vi "CSM - Revert Arguments-Safe String.vi"(2 "Safe Argument String":string="eaasdf->fqwvrf", 4 "Force Convert (F)":bool) -> (7 "Origin Argument String":string)   [LabVIEW 2017, in "Communicable State Machine.lvlib"]
doc: "Converts the %Hex format CSM keywords in the safe string argument back to the original format.\n\n- When <b>Force Convert (F)</b> is FALSE, conversion is performed only if the argument type tag is `SAFESTR`.\n- When <b>Force Convert (F)</b> is TRUE, conversion is performed regardless of the argument type tag.\n\n\n> [!NOTE] <b>CSM Message Keywords</b>\n>\n> The following are CSM message keywords: `->`, `->|`, `-@`, `-&`, `<-`, `\\r`, `\\n`, `//`, `>>`, `>>>`, `>>>>`, `;`, `,`.\n\n\n> [!NOTE] <b>CSM Safe String Argument</b>\n>\n> To pass arbitrary strings in CSM arguments without disrupting message parsing, CSM has a built-in Safe-String encoding/decoding scheme. The argument type string is SAFESTR. The conversion process is as follows:\n> 1. Scan the input string. If any CSM keywords, such as `->`, `;`, `\\r` appear, replace them with `%Hex` escape sequences.\n> 2. Obtain the argument in the form `<SAFESTR> escaped string`, which can be safely embedded in the state string without disrupting CSM message parsing.\n\n\n<b>Reference Example</b>: `[CSM-Example]\\0. Base Concepts\\4.3 Arguments - Safe Arguments if it contains key words of CSM.vi`.\n\n-- <b>Controls</b> --\n- <b>Safe Argument String</b>: Safe string argument.\n- <b>Force Convert (F)</b>: Force conversion, even if the argument type tag is not `SAFESTR`.\n\n-- <b>Indicators</b> --\n- <b>Origin Argument String</b>: String argument."
uses:
  Communicable State Machine.lvlib
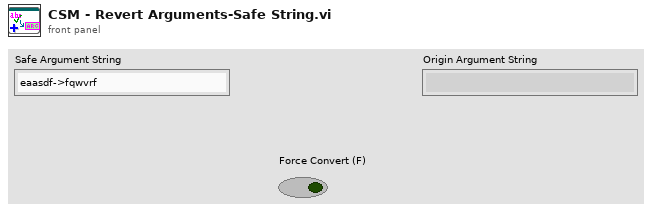
[diagram p1: front panel]
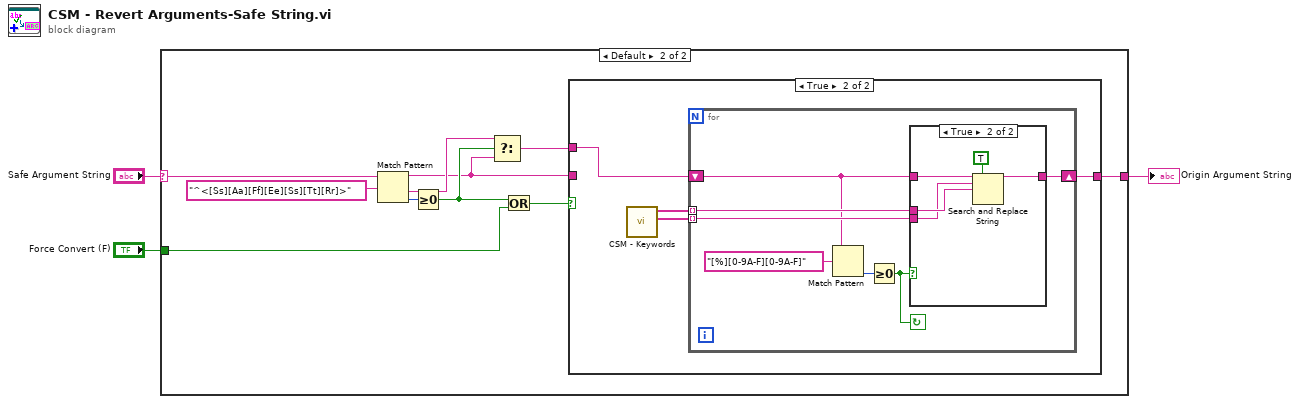
[diagram p0: block diagram]
diagram:
  n1 = case shown="Default" "Safe Argument String" {
    selector: "Safe Argument String" -> [w4 w11]
    tunnel: [w4 w14] -> w2
    tunnel: "Force Convert (F)" -> [_ w9]
    frame "" {
    }
    frame Default {
      n2 = Match Pattern(string=w11, regular expression="^<[Ss][Aa][Ff][Ee][Ss][Tt][Rr]>") -> (before substring=w6:string, after substring=w7:string, offset past match=w12:i32)  [unwired: 1 in, 1 out]
      n3 = Greater Or Equal To 0?(x=w12) -> (x >= 0?=w8:bool)
      n4 = Select(t=w7, s=w8, f=w6) -> (s? t:f=w5:string)
      n5 = Or(x=w8, y=w9) -> (x .or. y?=w10:bool)
      n6 = case shown="True" w10 {
        tunnel: [w15 w19] -> w14
        tunnel: w6 -> [w15 _]
        tunnel: w5 -> [_ w16]
        frame False {
        }
        frame True {
          n7 = call "CSM - Keywords.vi"() -> ("Keywords (%Hex Format)"=w18:string[], "Keywords"=w17:string[])  [unwired: 10 in]
          n8 = for {
            shift-right: [w26] -> w19
            shift-left: w16 -> [w23]
            tunnel: w17 -> [w25] mode=indexing
            tunnel: w18 -> [w24] mode=indexing
            stop <- w20 continue-if-true
            n9 = Match Pattern(string=w23, regular expression="[%][0-9A-F][0-9A-F]") -> (offset past match=w21:i32)  [unwired: 1 in, 3 out]
            n10 = Greater Or Equal To 0?(x=w21) -> (x >= 0?=w20:bool)
            n11 = case shown="True" w20 {
              tunnel: [w27 w31] -> w26
              tunnel: w25 -> [_ w30]
              tunnel: w24 -> [_ w29]
              tunnel: w23 -> [w27 w28]
              frame False {
              }
              frame True {
                n12 = Search and Replace String(replace all?=TRUE ("replace all? (F)"), input string=w28, search string=w29, replace string=w30) -> (result string=w31:string)  [unwired: 4 in, 3 out]
              }
            }
          }
        }
      }
    }
  }
  "Origin Argument String" <- w2
